vi "OwnCompat20261012_Native_SetControlPosition.vi"() -> ()   [LabVIEW 2024]
panel:
  out "error out":errorcluster caption="错误输出"
  in  "y":i16=100
  in  "x":i16=100
  in  "control_id":u32
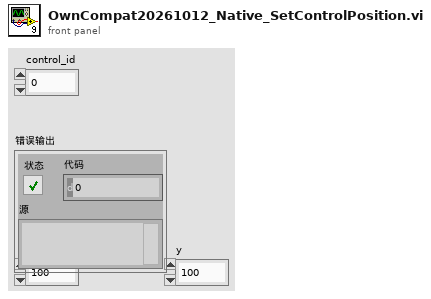
[diagram p1: front panel]
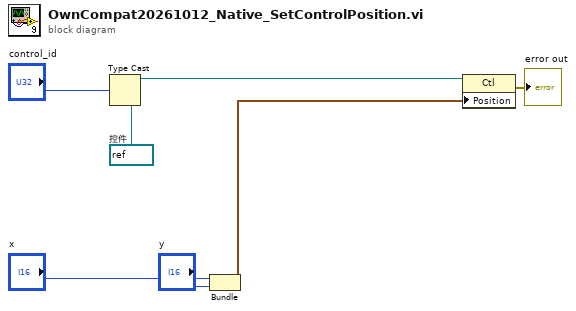
[diagram p0: block diagram]
diagram:
  w6 = refnum<vi> refnum  # 控件
  n1 = Type Cast ("强制类型转换")(type=w6, x="control_id") -> (*(type *) &x=w3:refnum<vi>)
  n2 = Bundle ("捆绑")("x"="x", "y"="y") -> (w2:cluster{"x":i16, "y":i16})  [unwired: 1 in]
  n3 = property on="属性节点" class="Ctl"(reference=w3, "Position"=w2) -> (error out=→"error out":errorcluster)  [unwired: 1 in, 1 out]
